vi "Select OPC UA Class.vi"(8 "error in":errorcluster, 10 "Class Path":path=path "C:/GitHub/OOP Template/HAL/Concrete") -> (0 "error out":errorcluster, 3 "Object":refnum<class>)   [LabVIEW 2025, in "Abstract.lvclass"]
uses:
  Abstract.lvclass
  Submodule EOL/Submodule EOL.lvclass/Submodule EOL.ctl
  Abstract.lvclass/Abstract.ctl
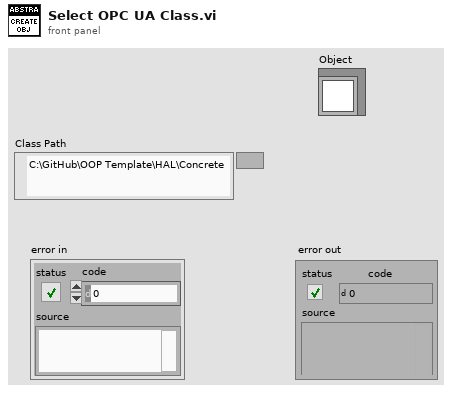
[diagram p1: front panel]
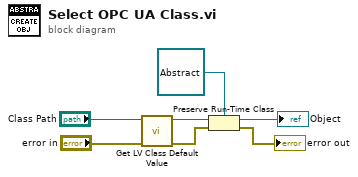
[diagram p0: block diagram]
diagram:
  n1 = call <vilib>:"Get LV Class Default Value.vi"("error in (no error)"="error in", "class path"="Class Path") -> ("error out"=w6:errorcluster, "object"=w2:refnum<class>)  [unwired: 8 in]
  n2 = Preserve Run-Time Class(object in=w2, error in=w6, 2:refnum<class "Abstract.lvclass"> refnum ("Abstract")) -> (object out=→"Object":refnum<class "Abstract.lvclass">, error out=→"error out":errorcluster)
